vi "main-thermocouple-logger.vi"() -> ()   [LabVIEW 2024]
uses:
  controls/adam-5000-serial-settings.ctl
  controls/adam-5000-cmd-response.ctl
  controls/state-enum.ctl
  sub-vi/csv-file-logging/filepath-selection.ctl
  controls/adam-5000-all-chassis-data.ctl
  controls/adam-5000-all-module-datas.ctl
  controls/digital-output-cluster.ctl
  controls/digitial-input-cluster.ctl
  controls/analog-output-cluster.ctl
  controls/analog-input-cluster.ctl
  controls/thermocouple-input-cluster.ctl
  controls/adam-5000-chassis-cmd-ack.ctl
  controls/adam-5000-chassis-module-types.ctl
  controls/adam-5000-DO-user-input.ctl
  controls/adam-5000-status-indicator-references.ctl
panel:
  out "T12":dbl
  out "T11":dbl
  out "T6 (Airgap)":dbl
  out "T5 (Ambi)":dbl
  in  "TC5:8 Zero Point Offset":cluster{"T5":dbl, "T6":dbl, "T7":dbl, "T8":dbl}
  in  "TC1:4 Zero point offset":cluster{"T1":dbl, "T2":dbl, "T3":dbl, "T4":dbl}
  in  "Calibration":bool
  in  "clear-graphs":bool
  out "Thermocouples 5-8":T1(graph)
  out "Thermocouples 1-4":T1(graph)
  out "T10":dbl
  out "T9":dbl
  out "T8":dbl
  out "T7":dbl
  out "T4":dbl
  out "T3":dbl
  out "T2":dbl
  out "T1":dbl
  out "Hz":dbl format="%_3g"
  in  "Sample Rate (Hz)":dbl=1.0 min=0.0001 max=4.0 format="%#_4g"
  out "Logged Data String":string
  in  "CSV Data Headings":string="time (s),T1,T2,T3,T4,T5(Ambi),T6(Airgap),T7, T8, T9, T10, T11, T12"
  out "log-elapsed time":dbl format="%.2f"
  out "log start time":u32
  out "File Open":bool
  out "Log Filepath":path
  in  "Log Filepath Selection":T2={"Log Filepath Source"=enum."Application Relative (Auto)", "Log File Path (Manual)"=path "C:/Users/iwheard/Documents/0000-labview/adam5000-generic-controller/data", "Log File Folder Name"="data", "log file name"="log", "Include Date in Filename"=TRUE, "Include Time in Filename"=TRUE}
  out "Logging Active":bool
  out "Error Detected":bool
  in  "Reset":bool
  out "ADAM Connected":bool
  in  "Stop ADAM":bool
  in  "Start Logging":bool
  out "Program State":T3
  in  "Start ADAM":bool
  out "cmd-response":T5
  out "Status Indicators":T6
  in  "Debug Mode":bool
  in  "Chassis Settings":T7={"VISA resource name"="COM3", "baud rate (19200)"=19200, "Chassis ID"=1}
  out "Loop Time (mS)":u32
  out "Loop Counter":i32
  out "error":errorcluster
  in  "exit":bool
  # "ADAM 5000 Controller"
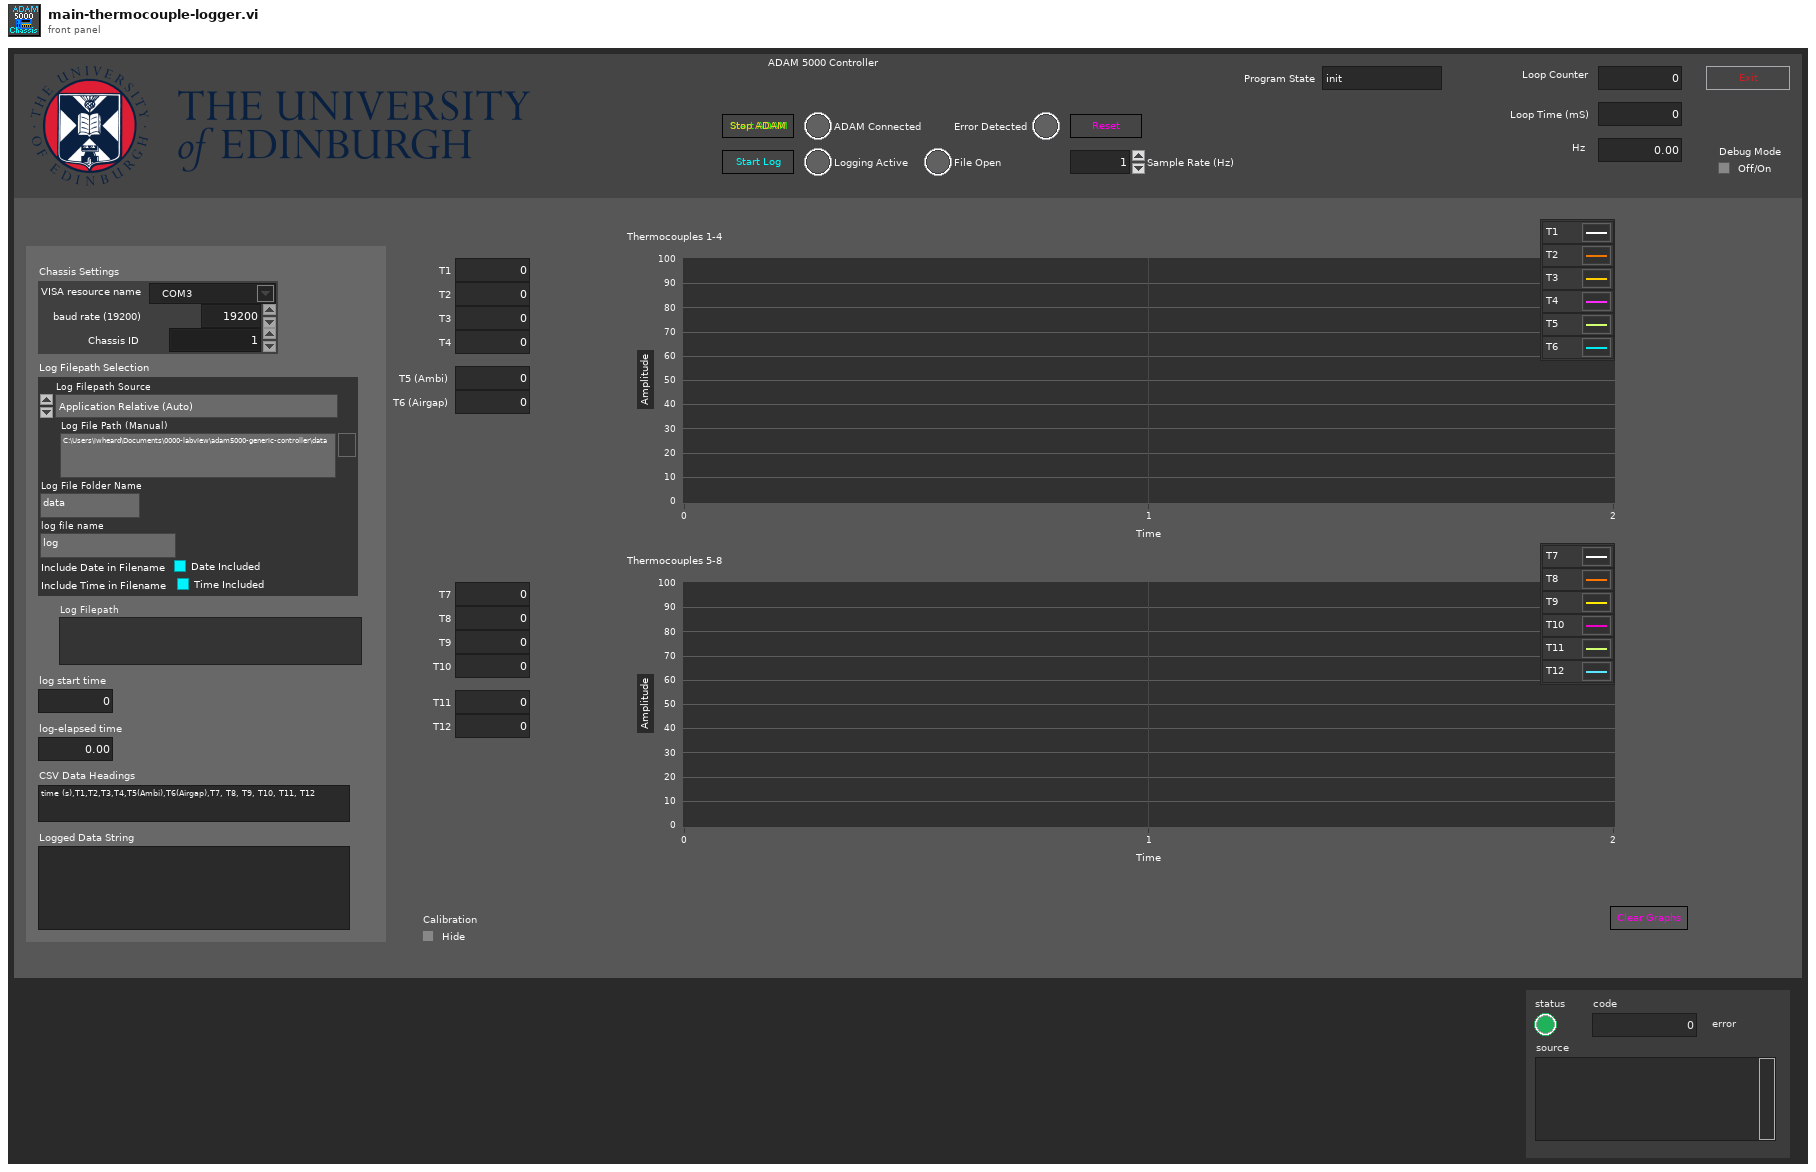
[diagram p1: front panel]
types:
  T1 = cluster{"TC0":dbl, "TC1":dbl, "TC2":dbl, "TC3":dbl, "TC4":dbl, "TC5":dbl, "TC6":dbl}
  T2 = typedef "filepath-selection.ctl" = cluster{"Log Filepath Source":enum16{"Application Relative (Auto)", "VI Relative (Auto)", "Complete Path (Manual)"}, "Log File Path (Manual)":path, "Log File Folder Name":string, "log file name":string, "Include Date in Filename":bool, "Include Time in Filename":bool}
  T3 = typedef "state-enum.ctl" = enum16{"init", "wait", "manual", "start", "run", "reset", "stop", "exit"}
  T4 = typedef "adam-5000-cmd-response.ctl" = cluster{"cmd string":string, "response":string}
  T5 = cluster{"cmd-response:0":T4, "cmd-response:1":T4, "cmd-response:2":T4, "cmd-response:3":T4, "cmd-response:4":T4, "cmd-response:5":T4, "cmd-response:6":T4, "cmd-response:7":T4}
  T6 = cluster{"status-indicator:0":cluster{"Sampling":bool, "Ack":bool}, "status-indicator:1":cluster{"Sampling":bool, "Ack":bool}, "status-indicator:2":cluster{"Sampling":bool, "Ack":bool}, "status-indicator:3":cluster{"Sampling":bool, "Ack":bool}, "status-indicator:4":cluster{"Sampling":bool, "Ack":bool}, "status-indicator:5":cluster{"Sampling":bool, "Ack":bool}, "status-indicator:6":cluster{"Sampling":bool, "Ack":bool}, "status-indicator:7":cluster{"Sampling":bool, "Ack":bool}}
  T7 = typedef "adam-5000-serial-settings.ctl" = cluster{"VISA resource name":refnum<visa-resource-name>, "baud rate (19200)":u32, "Chassis ID":u8}
  T8 = enum16{"Digital Output", "Digital Input", "Analog Output", "Analog Input", "Thermocouple", "Power Relay", "empty"}
  T9 = typedef "adam-5000-chassis-module-types.ctl" = cluster{"Slot 0: Module Type":enum16{"Digital Output", "Digital Input", "Analog Output", "Analog Input", "Thermocouple", "Power Relay", "empty"}, "Slot 1: Module Type":enum16{"Digital Output", "Digital Input", "Analog Output", "Analog Input", "Thermocouple", "Power Relay", "empty"}, "Slot 2: Module Type":enum16{"Digital Output", "Digital Input", "Analog Output", "Analog Input", "Thermocouple", "Power Relay", "empty"}, "Slot 3: Module Type":enum16{"Digital Output", "Digital Input", "Analog Output", "Analog Input", "Thermocouple", "Power Relay", "empty"}, "Slot 4: Module Type":enum16{"Digital Output", "Digital Input", "Analog Output", "Analog Input", "Thermocouple", "Power Relay", "empty"}, "Slot 5: Module Type":enum16{"Digital Output", "Digital Input", "Analog Output", "Analog Input", "Thermocouple", "Power Relay", "empty"}, "Slot 6: Module Type":enum16{"Digital Output", "Digital Input", "Analog Output", "Analog Input", "Thermocouple", "Power Relay", "empty"}, "Slot 7: Module Type":enum16{"Digital Output", "Digital Input", "Analog Output", "Analog Input", "Thermocouple", "Power Relay", "empty"}}
  T10 = typedef "adam-5000-chassis-cmd-ack.ctl" = cluster{"cmd-response:0":T4, "cmd-response:1":T4, "cmd-response:2":T4, "cmd-response:3":T4, "cmd-response:4":T4, "cmd-response:5":T4, "cmd-response:6":T4, "cmd-response:7":T4}
  T11 = typedef "adam-5000-all-chassis-data.ctl" = cluster{"slot:0":T12, "slot:1":T12, "slot:2":T12, "slot:3":T12, "slot:4":T12, "slot:5":T12, "slot:6":T12, "slot:7":T12}
  T12 = typedef "adam-5000-all-module-datas.ctl" = cluster{"Digital Outputs":T13, "Digital Inputs":T14, "Analog Outputs":T15, "Analog Inputs":T16, "Thermocouple Inputs (degC)":T17}
  T13 = typedef "digital-output-cluster.ctl" = cluster{"DO0":bool, "DO1":bool, "DO2":bool, "DO3":bool, "DO4":bool, "DO5":bool, "DO6":bool, "DO7":bool}
  T14 = typedef "digitial-input-cluster.ctl" = cluster{"DI0":bool, "DI1":bool, "DI2":bool, "DI3":bool, "DI4":bool, "DI5":bool, "DI6":bool, "DI7":bool}
  T15 = typedef "analog-output-cluster.ctl" = cluster{"AO0":dbl, "AO1":dbl, "AO2":dbl, "AO3":dbl}
  T16 = typedef "analog-input-cluster.ctl" = cluster{"AI0":dbl, "AI1":dbl, "AI2":dbl, "AI3":dbl, "AI4":dbl, "AI5":dbl, "AI6":dbl, "AI7":dbl}
  T17 = typedef "thermocouple-input-cluster.ctl" = cluster{"TC0":dbl, "TC1":dbl, "TC2":dbl, "TC3":dbl, "TC4":dbl, "TC5":dbl, "TC6":dbl}
  T18 = enum8{"Enabled", "Disabled", "Disabled and Grayed Out"}
  T19 = typedef "adam-5000-status-indicator-references.ctl" = cluster{"status-indicator:0":refnum<vi>, "status-indicator:1":refnum<vi>, "status-indicator:2":refnum<vi>, "status-indicator:3":refnum<vi>, "status-indicator:4":refnum<vi>, "status-indicator:5":refnum<vi>, "status-indicator:6":refnum<vi>, "status-indicator:7":refnum<vi>}
  T20 = typedef "adam-5000-DO-user-input.ctl" = cluster{"0:Digital Outputs":T13, "1:Digital Outputs":T13, "2:Digital Outputs":T13, "3:Digital Outputs":T13, "4:Digital Outputs":T13, "5:Digital Outputs":T13, "6:Digital Outputs":T13, "7:Digital Outputs":T13}
  T21 = cluster{"TC0":dbl, "TC1":dbl, "TC2":dbl, "TC3":dbl, "TC4":dbl, "TC5":dbl, "TC6":dbl}[]
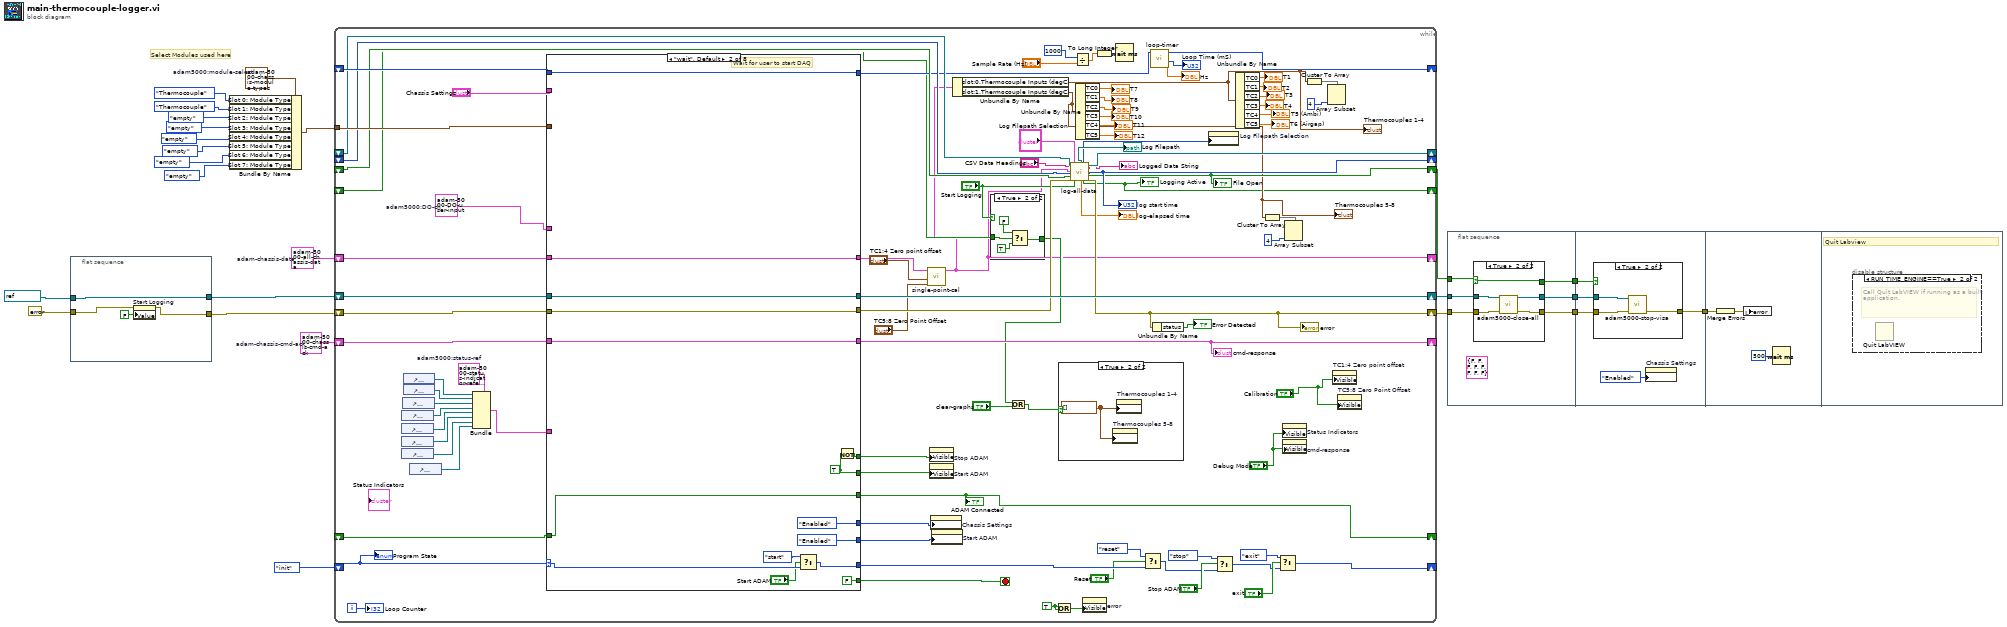
[diagram p0: block diagram]
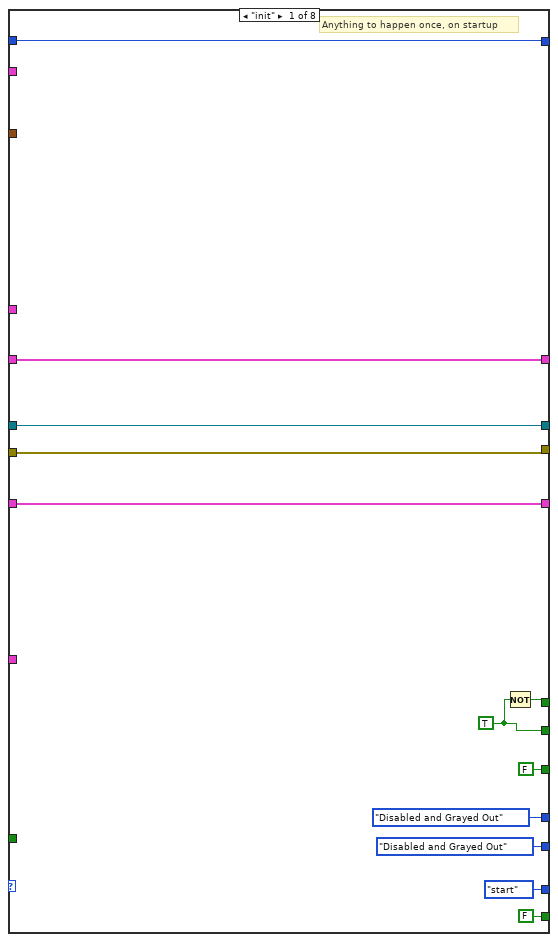
[diagram p7: hidden frame]
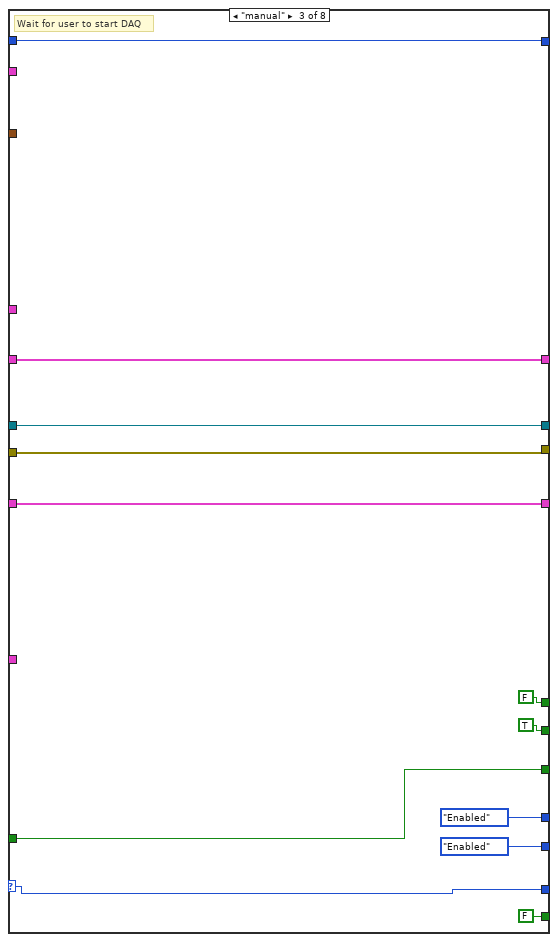
[diagram p8: hidden frame]
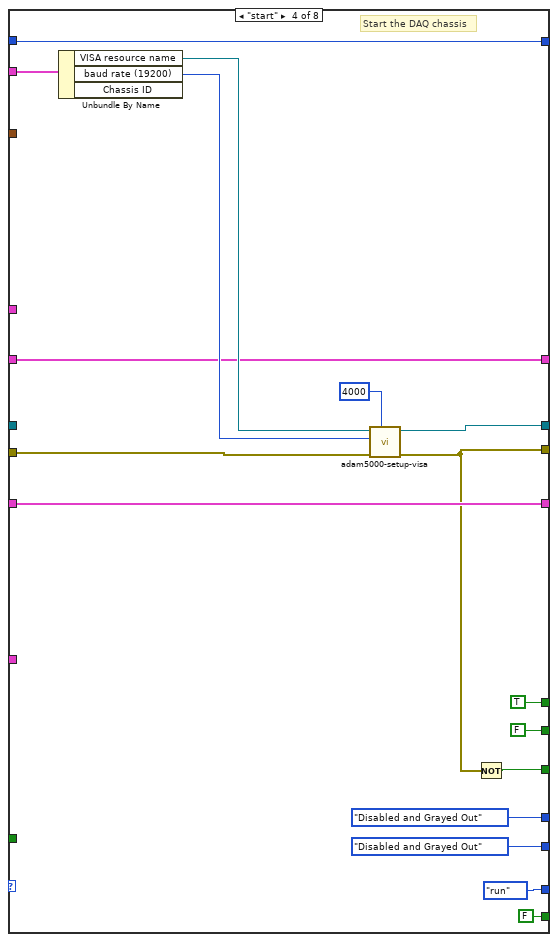
[diagram p9: hidden frame]
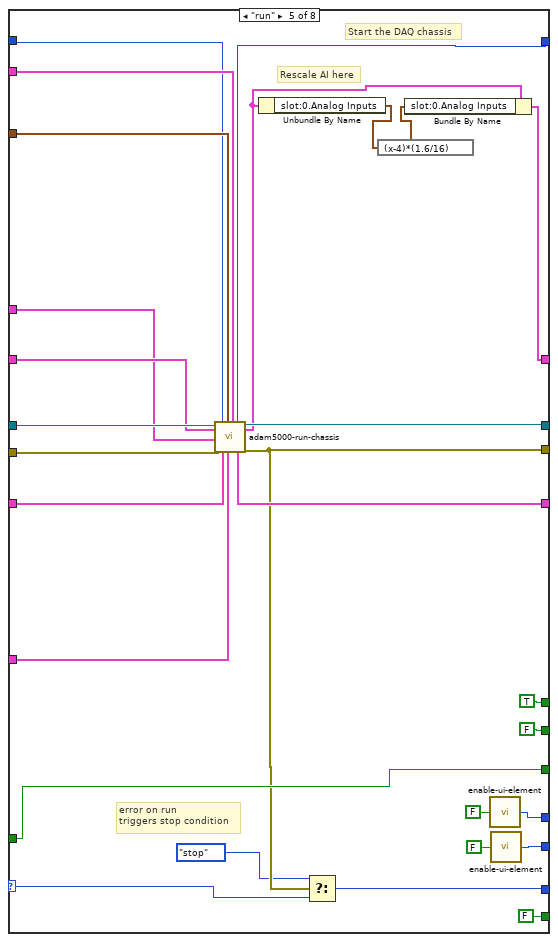
[diagram p10: hidden frame]
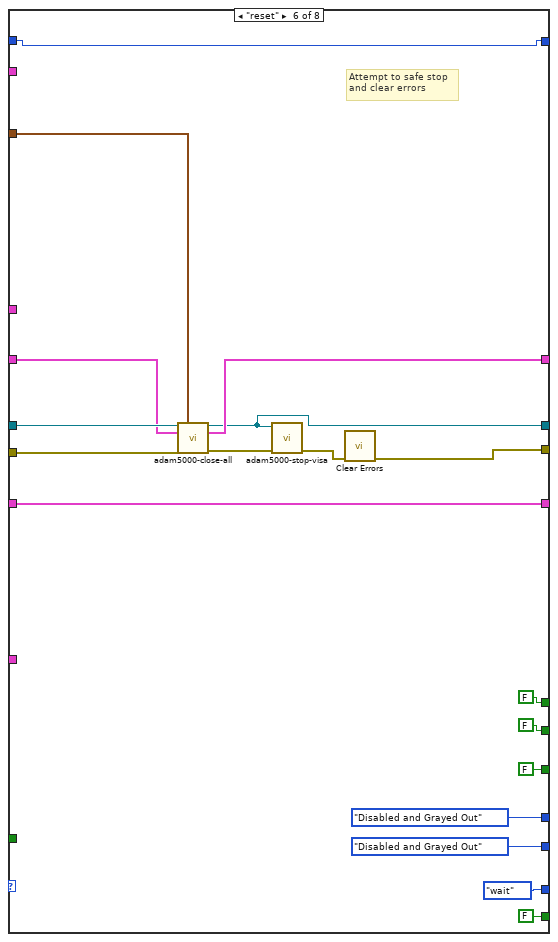
[diagram p11: hidden frame]
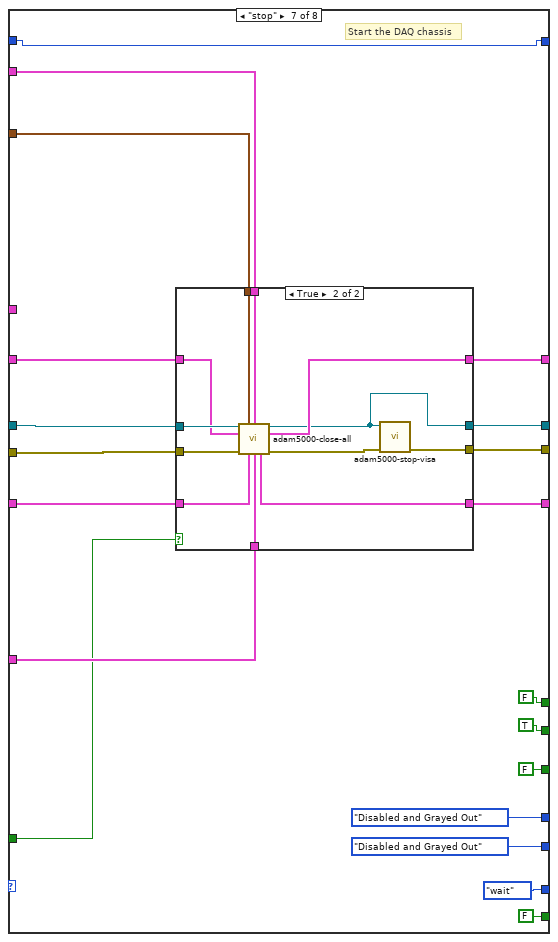
[diagram p12: hidden frame]
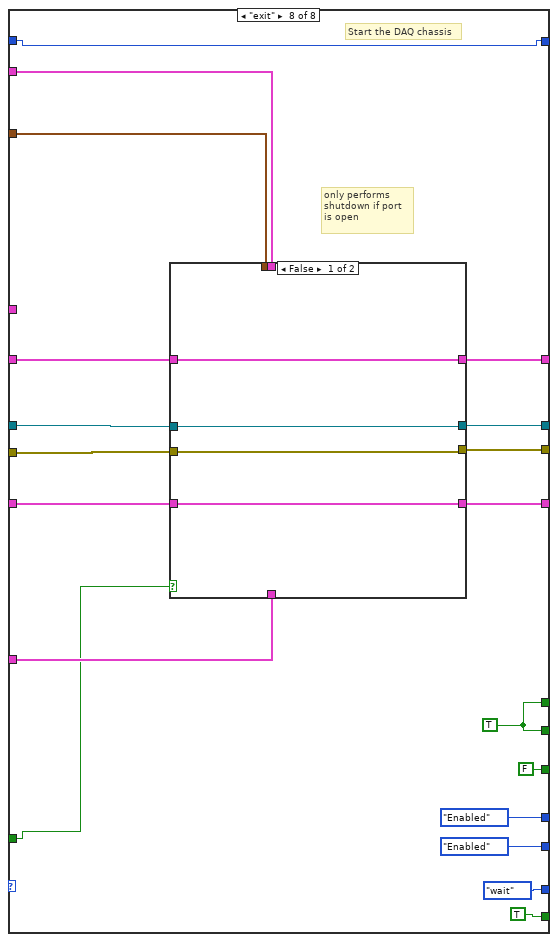
[diagram p14: hidden frame]
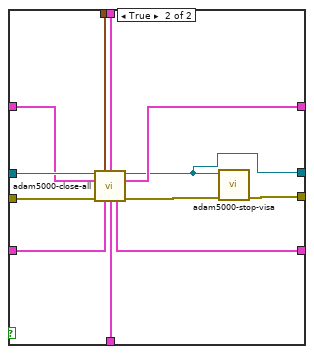
[diagram p15: hidden frame]
diagram:
  w16 = T9 {"Slot 0: Module Type"=enum."Digital Output", "Slot 1: Module Type"=enum."Digital Output", "Slot 2: Module Type"=enum."Digital Output", "Slot 3: Module Type"=enum."Digital Output", "Slot 4: Module Type"=enum."Digital Output", "Slot 5: Module Type"=enum."Digital Output", "Slot 6: Module Type"=enum."Digital Output", "Slot 7: Module Type"=enum."Digital Output"}  # adam5000:module-select
  w21 = T10 {"cmd-response:0"={"cmd string"="", "response"=""}, "cmd-response:1"={"cmd string"="", "response"=""}, "cmd-response:2"={"cmd string"="", "response"=""}, "cmd-response:3"={"cmd string"="", "response"=""}, "cmd-response:4"={"cmd string"="", "response"=""}, "cmd-response:5"={"cmd string"="", "response"=""}, "cmd-response:6"={"cmd string"="", "response"=""}, "cmd-response:7"={"cmd string"="", "response"=""}}  # adam-chassis-cmd-ack
  w22 = T11 {"slot:0"={"Digital Outputs"={"DO0"=FALSE, "DO1"=FALSE, "DO2"=FALSE, "DO3"=FALSE, "DO4"=FALSE, "DO5"=FALSE, "DO6"=FALSE, "DO7"=FALSE}, "Digital Inputs"={"DI0"=FALSE, "DI1"=FALSE, "DI2"=FALSE, "DI3"=FALSE, "DI4"=FALSE, "DI5"=FALSE, "DI6"=FALSE, "DI7"=FALSE}, "Analog Outputs"={"AO0"=0.0, "AO1"=0.0, "AO2"=0.0, "AO3"=0.0}, "Analog Inputs"={"AI0"=0.0, "AI1"=0.0, "AI2"=0.0, "AI3"=0.0, "AI4"=0.0, "AI5"=0.0, "AI6"=0.0, "AI7"=0.0}, "Thermocouple Inputs (degC)"={"TC0"=0.0, "TC1"=0.0, "TC2"=0.0, "TC3"=0.0, "TC4"=0.0, "TC5"=0.0, "TC6"=0.0}}, "slot:1"={"Digital Outputs"={"DO0"=FALSE, "DO1"=FALSE, "DO2"=FALSE, "DO3"=FALSE, "DO4"=FALSE, "DO5"=FALSE, "DO6"=FALSE, "DO7"=FALSE}, "Digital Inputs"={"DI0"=FALSE, "DI1"=FALSE, "DI2"=FALSE, "DI3"=FALSE, "DI4"=FALSE, "DI5"=FALSE, "DI6"=FALSE, "DI7"=FALSE}, "Analog Outputs"={"AO0"=0.0, "AO1"=0.0, "AO2"=0.0, "AO3"=0.0}, "Analog Inputs"={"AI0"=0.0, "AI1"=0.0, "AI2"=0.0, "AI3"=0.0, "AI4"=0.0, "AI5"=0.0, "AI6"=0.0, "AI7"=0.0}, "Thermocouple Inputs (degC)"={"TC0"=0.0, "TC1"=0.0, "TC2"=0.0, "TC3"=0.0, "TC4"=0.0, "TC5"=0.0, "TC6"=0.0}}, "slot:2"={"Digital Outputs"={"DO0"=FALSE, "DO1"=FALSE, "DO2"=FALSE, "DO3"=FALSE, "DO4"=FALSE, "DO5"=FALSE, "DO6"=FALSE, "DO7"=FALSE}, "Digital Inputs"={"DI0"=FALSE, "DI1"=FALSE, "DI2"=FALSE, "DI3"=FALSE, "DI4"=FALSE, "DI5"=FALSE, "DI6"=FALSE, "DI7"=FALSE}, "Analog Outputs"={"AO0"=0.0, "AO1"=0.0, "AO2"=0.0, "AO3"=0.0}, "Analog Inputs"={"AI0"=0.0, "AI1"=0.0, "AI2"=0.0, "AI3"=0.0, "AI4"=0.0, "AI5"=0.0, "AI6"=0.0, "AI7"=0.0}, "Thermocouple Inputs (degC)"={"TC0"=0.0, "TC1"=0.0, "TC2"=0.0, "TC3"=0.0, "TC4"=0.0, "TC5"=0.0, "TC6"=0.0}}, "slot:3"={"Digital Outputs"={"DO0"=FALSE, "DO1"=FALSE, "DO2"=FALSE, "DO3"=FALSE, "DO4"=FALSE, "DO5"=FALSE, "DO6"=FALSE, "DO7"=FALSE}, "Digital Inputs"={"DI0"=FALSE, "DI1"=FALSE, "DI2"=FALSE, "DI3"=FALSE, "DI4"=FALSE, "DI5"=FALSE, "DI6"=FALSE, "DI7"=FALSE}, "Analog Outputs"={"AO0"=0.0, "AO1"=0.0, "AO2"=0.0, "AO3"=0.0}, "Analog Inputs"={"AI0"=0.0, "AI1"=0.0, "AI2"=0.0, "AI3"=0.0, "AI4"=0.0, "AI5"=0.0, "AI6"=0.0, "AI7"=0.0}, "Thermocouple Inputs (degC)"={"TC0"=0.0, "TC1"=0.0, "TC2"=0.0, "TC3"=0.0, "TC4"=0.0, "TC5"=0.0, "TC6"=0.0}}, "slot:4"={"Digital Outputs"={"DO0"=FALSE, "DO1"=FALSE, "DO2"=FALSE, "DO3"=FALSE, "DO4"=FALSE, "DO5"=FALSE, "DO6"=FALSE, "DO7"=FALSE}, "Digital Inputs"={"DI0"=FALSE, "DI1"=FALSE, "DI2"=FALSE, "DI3"=FALSE, "DI4"=FALSE, "DI5"=FALSE, "DI6"=FALSE, "DI7"=FALSE}, "Analog Outputs"={"AO0"=0.0, "AO1"=0.0, "AO2"=0.0, "AO3"=0.0}, "Analog Inputs"={"AI0"=0.0, "AI1"=0.0, "AI2"=0.0, "AI3"=0.0, "AI4"=0.0, "AI5"=0.0, "AI6"=0.0, "AI7"=0.0}, "Thermocouple Inputs (degC)"={"TC0"=0.0, "TC1"=0.0, "TC2"=0.0, "TC3"=0.0, "TC4"=0.0, "TC5"=0.0, "TC6"=0.0}}, "slot:5"={"Digital Outputs"={"DO0"=FALSE, "DO1"=FALSE, "DO2"=FALSE, "DO3"=FALSE, "DO4"=FALSE, "DO5"=FALSE, "DO6"=FALSE, "DO7"=FALSE}, "Digital Inputs"={"DI0"=FALSE, "DI1"=FALSE, "DI2"=FALSE, "DI3"=FALSE, "DI4"=FALSE, "DI5"=FALSE, "DI6"=FALSE, "DI7"=FALSE}, "Analog Outputs"={"AO0"=0.0, "AO1"=0.0, "AO2"=0.0, "AO3"=0.0}, "Analog Inputs"={"AI0"=0.0, "AI1"=0.0, "AI2"=0.0, "AI3"=0.0, "AI4"=0.0, "AI5"=0.0, "AI6"=0.0, "AI7"=0.0}, "Thermocouple Inputs (degC)"={"TC0"=0.0, "TC1"=0.0, "TC2"=0.0, "TC3"=0.0, "TC4"=0.0, "TC5"=0.0, "TC6"=0.0}}, "slot:6"={"Digital Outputs"={"DO0"=FALSE, "DO1"=FALSE, "DO2"=FALSE, "DO3"=FALSE, "DO4"=FALSE, "DO5"=FALSE, "DO6"=FALSE, "DO7"=FALSE}, "Digital Inputs"={"DI0"=FALSE, "DI1"=FALSE, "DI2"=FALSE, "DI3"=FALSE, "DI4"=FALSE, "DI5"=FALSE, "DI6"=FALSE, "DI7"=FALSE}, "Analog Outputs"={"AO0"=0.0, "AO1"=0.0, "AO2"=0.0, "AO3"=0.0}, "Analog Inputs"={"AI0"=0.0, "AI1"=0.0, "AI2"=0.0, "AI3"=0.0, "AI4"=0.0, "AI5"=0.0, "AI6"=0.0, "AI7"=0.0}, "Thermocouple Inputs (degC)"={"TC0"=0.0, "TC1"=0.0, "TC2"=0.0, "TC3"=0.0, "TC4"=0.0, "TC5"=0.0, "TC6"=0.0}}, "slot:7"={"Digital Outputs"={"DO0"=FALSE, "DO1"=FALSE, "DO2"=FALSE, "DO3"=FALSE, "DO4"=FALSE, "DO5"=FALSE, "DO6"=FALSE, "DO7"=FALSE}, "Digital Inputs"={"DI0"=FALSE, "DI1"=FALSE, "DI2"=FALSE, "DI3"=FALSE, "DI4"=FALSE, "DI5"=FALSE, "DI6"=FALSE, "DI7"=FALSE}, "Analog Outputs"={"AO0"=0.0, "AO1"=0.0, "AO2"=0.0, "AO3"=0.0}, "Analog Inputs"={"AI0"=0.0, "AI1"=0.0, "AI2"=0.0, "AI3"=0.0, "AI4"=0.0, "AI5"=0.0, "AI6"=0.0, "AI7"=0.0}, "Thermocouple Inputs (degC)"={"TC0"=0.0, "TC1"=0.0, "TC2"=0.0, "TC3"=0.0, "TC4"=0.0, "TC5"=0.0, "TC6"=0.0}}}  # adam-chassis-data
  # "Select Modules used here"
  n1 = flat-sequence {
    tunnel: [w27] -> w5
    tunnel: refnum<visa-resource-name> "COM8" ("VISA Refnum out") -> [w27]
    tunnel: errorcluster {"status"=FALSE, "code"=0, "source"=""} ("error in") -> [w26]
    tunnel: [w25] -> w3
    frame #0 {
      n2 = property on="Start Logging" class="Bool (strict)"(error in=w26, "Value"=FALSE ("Start Logging")) -> (error out=w25:errorcluster)  [unwired: 1 in, 1 out]
    }
  }
  n3 = Bundle By Name(cluster=w16, "Slot 0: Module Type"=T8."Thermocouple", "Slot 1: Module Type"=T8."Thermocouple", "Slot 2: Module Type"=T8."empty" ("Slot 1: Module Type"), "Slot 3: Module Type"=T8."empty" ("Slot 1: Module Type"), "Slot 4: Module Type"=T8."empty" ("Slot 1: Module Type"), "Slot 5: Module Type"=T8."empty" ("Slot 1: Module Type"), "Slot 6: Module Type"=T8."empty" ("Slot 1: Module Type"), "Slot 7: Module Type"=T8."empty" ("Slot 1: Module Type")) -> (w7:T9)
  n4 = while {
    shift-right: [w101] -> _
    shift-left: state-enum."init" ("state-enum") -> [w84]
    shift-right: [w67] -> _
    shift-left: _ -> [w105]
    shift-right: [w93] -> w20
    shift-left: w5 -> [w108]
    shift-right: [w71] -> w19
    shift-left: w3 -> [w107]
    shift-right: [w35] -> _
    shift-left: w22 -> [w104]
    shift-right: [w86] -> _
    shift-left: w21 -> [w103]
    shift-right: [w91] -> _
    shift-left: _ -> [w92]
    tunnel: w7 -> [w85]
    shift-right: [w59] -> w2
    shift-left: _ -> [w72]
    shift-right: [w60] -> _
    shift-left: _ -> [w73]
    shift-right: [w77] -> _
    shift-left: _ -> [w80]
    shift-right: [w43] -> _
    shift-left: _ -> [w39]
    i -> [w122]
    stop <- w94 stop-if-true
    w112 = T19 {"status-indicator:0"=refnum, "status-indicator:1"=refnum, "status-indicator:2"=refnum, "status-indicator:3"=refnum, "status-indicator:4"=refnum, "status-indicator:5"=refnum, "status-indicator:6"=refnum, "status-indicator:7"=refnum}  # adam5000:status-ref
    w58 = T20 {"0:Digital Outputs"={"DO0"=FALSE, "DO1"=FALSE, "DO2"=FALSE, "DO3"=FALSE, "DO4"=FALSE, "DO5"=FALSE, "DO6"=FALSE, "DO7"=FALSE}, "1:Digital Outputs"={"DO0"=FALSE, "DO1"=FALSE, "DO2"=FALSE, "DO3"=FALSE, "DO4"=FALSE, "DO5"=FALSE, "DO6"=FALSE, "DO7"=FALSE}, "2:Digital Outputs"={"DO0"=FALSE, "DO1"=FALSE, "DO2"=FALSE, "DO3"=FALSE, "DO4"=FALSE, "DO5"=FALSE, "DO6"=FALSE, "DO7"=FALSE}, "3:Digital Outputs"={"DO0"=FALSE, "DO1"=FALSE, "DO2"=FALSE, "DO3"=FALSE, "DO4"=FALSE, "DO5"=FALSE, "DO6"=FALSE, "DO7"=FALSE}, "4:Digital Outputs"={"DO0"=FALSE, "DO1"=FALSE, "DO2"=FALSE, "DO3"=FALSE, "DO4"=FALSE, "DO5"=FALSE, "DO6"=FALSE, "DO7"=FALSE}, "5:Digital Outputs"={"DO0"=FALSE, "DO1"=FALSE, "DO2"=FALSE, "DO3"=FALSE, "DO4"=FALSE, "DO5"=FALSE, "DO6"=FALSE, "DO7"=FALSE}, "6:Digital Outputs"={"DO0"=FALSE, "DO1"=FALSE, "DO2"=FALSE, "DO3"=FALSE, "DO4"=FALSE, "DO5"=FALSE, "DO6"=FALSE, "DO7"=FALSE}, "7:Digital Outputs"={"DO0"=FALSE, "DO1"=FALSE, "DO2"=FALSE, "DO3"=FALSE, "DO4"=FALSE, "DO5"=FALSE, "DO6"=FALSE, "DO7"=FALSE}}  # adam5000:DO-ch
    w95 = TRUE ("Debug Mode")
    n5 = control-ref of="status-indicator:4"() -> (w116:refnum<vi>)
    n6 = control-ref of="status-indicator:5"() -> (w115:refnum<vi>)
    n7 = control-ref of="status-indicator:3"() -> (w117:refnum<vi>)
    n8 = control-ref of="status-indicator:6"() -> (w114:refnum<vi>)
    n9 = control-ref of="status-indicator:2"() -> (w118:refnum<vi>)
    n10 = control-ref of="status-indicator:0"() -> (w120:refnum<vi>)
    n11 = control-ref of="status-indicator:1"() -> (w119:refnum<vi>)
    n12 = control-ref of="status-indicator:7"() -> (w113:refnum<vi>)
    n13 = Bundle(cluster=w112, "status-indicator:0"=w120, "status-indicator:1"=w119, "status-indicator:2"=w118, "status-indicator:3"=w117, "status-indicator:4"=w116, "status-indicator:5"=w115, "status-indicator:6"=w114, "status-indicator:7"=w113) -> (w102:T19)
    n14 = case shown="\"wait\", Default" w84 {
      selector: w84 -> [_ w153 w163 _ w197 _ _ _]
      tunnel: [state-enum."start" ("state-enum") w154 w163 state-enum."run" ("state-enum") w198 state-enum."wait" ("state-enum") state-enum."wait" ("state-enum") state-enum."wait" ("state-enum")] -> w89
      tunnel: [T18."Disabled and Grayed Out" ("Disabled") T18."Enabled" ("Disabled") T18."Enabled" ("Disabled") T18."Disabled and Grayed Out" ("Disabled") w187 T18."Disabled and Grayed Out" ("Disabled") T18."Disabled and Grayed Out" ("Disabled") T18."Enabled" ("Disabled")] -> w110
      tunnel: [T18."Disabled and Grayed Out" ("Disabled") T18."Enabled" ("Disabled") T18."Enabled" ("Disabled") T18."Disabled and Grayed Out" ("Disabled") w185 T18."Disabled and Grayed Out" ("Disabled") T18."Disabled and Grayed Out" ("Disabled") T18."Enabled" ("Disabled")] -> w109
      tunnel: w108 -> [w137 w150 w165 _ w212 w221 w247 w282]
      tunnel: [w137 w150 w165 w182 w210 w215 w237 w270] -> w93
      tunnel: w107 -> [w136 w149 w164 w181 w211 w220 w246 w281]
      tunnel: [w136 w149 w164 w171 w196 w224 w236 w271] -> w70
      tunnel: "Chassis Settings" -> [_ _ _ w180 w209 _ w244 w279]
      tunnel: w85 -> [_ _ _ _ w208 w217 w245 w280]
      tunnel: w105 -> [w135 w147 w162 w175 w207 w226 w238 w273]
      tunnel: [w135 w147 w162 w175 w206 w226 w238 w273] -> w68
      tunnel: w104 -> [w134 w146 w161 w174 w205 w219 w243 w278]
      tunnel: w58 -> [_ _ _ _ w204 _ _ _]
      tunnel: w103 -> [w133 w145 w160 w173 w203 w225 w241 w276]
      tunnel: w102 -> [_ _ _ _ w202 _ w240 w275]
      tunnel: [w133 w145 w160 w173 w201 w225 w239 w274] -> w86
      tunnel: [w134 w146 w161 w174 w191 w218 w242 w277] -> w37
      tunnel: [FALSE FALSE FALSE FALSE FALSE FALSE FALSE TRUE] -> w94
      tunnel: [FALSE w143 w158 w170 w199 FALSE FALSE FALSE] -> w91
      tunnel: w92 -> [_ w143 w158 _ w199 _ w233 w268]
      tunnel: [w130 w141 TRUE ("Visible") FALSE ("Visible") FALSE ("Visible") FALSE ("Visible") TRUE ("Visible") w267] -> w83
      tunnel: [w129 w142 FALSE ("Visible") TRUE ("Visible") TRUE ("Visible") FALSE ("Visible") FALSE ("Visible") w267] -> w82
      frame "init" {
        w130 = TRUE ("Visible")
        # "Anything to happen once, on startup"
        n15 = Not(x=w130) -> (.not. x?=w129:bool)
      }
      frame "wait", Default {
        w141 = TRUE ("Visible")
        # "Wait for user to start DAQ"
        n16 = Select(t=state-enum."start" ("state-enum"), s="Start ADAM", f=w153) -> (s? t:f=w154:T3)
        n17 = Not(x=w141) -> (.not. x?=w142:bool)
      }
      frame "manual" {
        # "Wait for user to start DAQ"
      }
      frame "start" {
        # "Start the DAQ chassis"
        n18 = Unbundle By Name(w180) -> ("VISA resource name"=w179:refnum<visa-resource-name>, "baud rate (19200)"=w178:u32)  [unwired: 1 out]
        n19 = call "adam5000-setup-visa.vi"("timeout (10sec)"=u32 4000, "error in"=w181, "baud rate (19200)"=w178, "VISA Refnum in"=w179) -> ("error out"=w171:errorcluster, "VISA Refnum out"=w182:refnum<visa-resource-name>)  [unwired: 6 in]
        n20 = Not(x=w171) -> (.not. x?=w170:bool)
      }
      frame "run" {
        # "Rescale AI here"
        # "error on run\ntriggers stop condition"
        # "Start the DAQ chassis"
        n21 = call "adam5000-run-chassis.vi"("VISA Refnum In"=w212, "adam-chassis-all-data-in"=w205, "adam-chassis-all-DO-in"=w204, "error in"=w211, "loop-time-in"=w207, "adam-chassis-cmd-response-in"=w203, "adam-chassis-module-select-in"=w208, "adam5000:status-ref-in"=w202, "Chassis Settings"=w209) -> ("loop-time-out"=w206:u32, "adam-chassis-cmd-response-out"=w201:T10, "VISA Refnum Out"=w210:refnum<visa-resource-name>, "adam-chassis-all-data-out"=w192:T11, "error out"=w196:errorcluster)  [unwired: 5 in, 1 out]
        n22 = Unbundle By Name(w192) -> ("slot:0.Analog Inputs"=w190:T16)
        n23 = Select(t=state-enum."stop", s=w196, f=w197) -> (s? t:f=w198:T3)
        n24 = expression code="(x-4)*(1.6/16)"(w190) -> (w189:T16)
        n25 = Bundle By Name(cluster=w192, "slot:0.Analog Inputs"=w189) -> (w191:T11)
        n26 = call "enable-ui-element.vi"("Enable UI Element"=FALSE) -> ("UI Element State"=w187:T18)  [unwired: 8 in]
        n27 = call "enable-ui-element.vi"("Enable UI Element"=FALSE) -> ("UI Element State"=w185:T18)  [unwired: 8 in]
      }
      frame "reset" {
        # "Attempt to safe stop\nand clear errors"
        n28 = call "adam5000-close-all.vi"("VISA Refnum in"=w221, "adam5000:module-type-select"=w217, "adam5000:all-data-in"=w219, "error in (no error)"=w220) -> ("VISA Refnum out"=w215:refnum<visa-resource-name>, "adam5000:all-data-out"=w218:T11, "error out"=w222:errorcluster)  [unwired: 8 in, 1 out]
        n29 = call "adam5000-stop-visa.vi"("error in (no error)"=w222, "VISA resource in"=w215) -> ("error out"=w216:errorcluster)  [unwired: 9 in]
        n30 = call <vilib>:"Clear Errors.vi"("error in (no error)"=w216) -> ("error out"=w224:errorcluster)  [unwired: 5 in, 1 out]
      }
      frame "stop" {
        # "Start the DAQ chassis"
        n31 = case shown="True" w233 {
          tunnel: w247 -> [w252 w266]
          tunnel: w246 -> [w251 w265]
          tunnel: w245 -> [_ w264]
          tunnel: w244 -> [_ w263]
          tunnel: w243 -> [w254 w262]
          tunnel: [w254 w261] -> w242
          tunnel: w241 -> [w253 w260]
          tunnel: w240 -> [_ w259]
          tunnel: [w253 w258] -> w239
          tunnel: [w252 w257] -> w237
          tunnel: [w251 w255] -> w236
          frame False {
          }
          frame True {
            n32 = call "adam5000-close-all.vi"("VISA Refnum in"=w266, "adam5000:module-type-select"=w264, "Chassis Settings in"=w263, "adam5000:all-data-in"=w262, "error in (no error)"=w265, "adam-chassis-cmd-ack"=w260, "adam5000:status-ref"=w259) -> ("VISA Refnum out"=w257:refnum<visa-resource-name>, "adam5000:all-data-out"=w261:T11, "adam-chassis-cmd-response-out"=w258:T10, "error out"=w256:errorcluster)  [unwired: 5 in]
            n33 = call "adam5000-stop-visa.vi"("error in (no error)"=w256, "VISA resource in"=w257) -> ("error out"=w255:errorcluster)  [unwired: 9 in]
          }
        }
      }
      frame "exit" {
        w267 = TRUE ("Visible")
        # "only performs\nshutdown if port\nis open"
        # "Start the DAQ chassis"
        n34 = case shown="False" w268 {
          tunnel: w282 -> [w288 w301]
          tunnel: w281 -> [w287 w300]
          tunnel: w280 -> [_ w299]
          tunnel: w279 -> [_ w298]
          tunnel: w278 -> [w289 w297]
          tunnel: [w289 w296] -> w277
          tunnel: w276 -> [w286 w295]
          tunnel: w275 -> [_ w294]
          tunnel: [w286 w293] -> w274
          tunnel: [w287 w291] -> w271
          tunnel: [w288 w290] -> w270
          frame False {
          }
          frame True {
            n35 = call "adam5000-close-all.vi"("VISA Refnum in"=w301, "adam5000:module-type-select"=w299, "Chassis Settings in"=w298, "adam5000:all-data-in"=w297, "error in (no error)"=w300, "adam-chassis-cmd-ack"=w295, "adam5000:status-ref"=w294) -> ("VISA Refnum out"=w290:refnum<visa-resource-name>, "adam5000:all-data-out"=w296:T11, "adam-chassis-cmd-response-out"=w293:T10, "error out"=w292:errorcluster)  [unwired: 5 in]
            n36 = call "adam5000-stop-visa.vi"("error in (no error)"=w292, "VISA resource in"=w290) -> ("error out"=w291:errorcluster)  [unwired: 9 in]
          }
        }
      }
    }
    "cmd-response" <- w86
    "ADAM Connected" <- w91
    n37 = call "single-point-cal.vi"("TC5:8 Zero Point Offset"="TC5:8 Zero Point Offset", "TC1:4 Zero point offset"="TC1:4 Zero point offset", "adam5000:all-data-in"=w37) -> ("adam5000:all-data-out"=w35:T11)  [unwired: 8 in]
    n38 = property on="Stop ADAM" class="Bool"("Visible"=w82) -> ()  [unwired: 2 in, 2 out]
    n39 = property on="Start ADAM" class="Bool"("Visible"=w83) -> ()  [unwired: 2 in, 2 out]
    n40 = property on="Chassis Settings" class="Clust (strict)"("DisabledEnum"=w110) -> ()  [unwired: 2 in, 2 out]
    n41 = property on="Start ADAM" class="Bool"("DisabledEnum"=w109) -> ()  [unwired: 2 in, 2 out]
    n42 = Unbundle By Name(w35) -> ("slot:0.Thermocouple Inputs (degC)"=w45:T17, "slot:1.Thermocouple Inputs (degC)"=w44:T17)
    "Thermocouples 1-4" <- w45
    "Thermocouples 5-8" <- w44
    n43 = case shown="True" "Start Logging" {
      selector: "Start Logging" -> [w123 _]
      tunnel: w39 -> [_ w127]
      tunnel: [w123 w125] -> w38
      frame False {
      }
      frame True {
        n44 = Select(t=FALSE ("Visible"), s=w127, f=TRUE ("Visible")) -> (s? t:f=w125:bool)
      }
    }
    n45 = Or(x=w38, y="clear-graphs") -> (x .or. y?=w42:bool)
    n46 = Or(x=w95, y=w95) -> (x .or. y?=w121:bool)
    n47 = case shown="True" w42 {
      frame False {
      }
      frame True {
        w128 = T21 [] ("History Data")
        n48 = property on="Thermocouples 5-8" class="WFChart (strict)"("History Data"=w128) -> ()  [unwired: 2 in, 2 out]
        n49 = property on="Thermocouples 1-4" class="WFChart (strict)"("History Data"=w128) -> ()  [unwired: 2 in, 2 out]
      }
    }
    n50 = call "log-all-data.vi"("log-file-byte-stream"=w80, "CSV Data Headings"="CSV Data Headings", "adam5000:all-data-in"=w35, "log-start-time(mS)"=w73, "file open?"=w72, "error in (no error)"=w70, "Log Filepath Selection"="Log Filepath Selection", "Start Logging"="Start Logging") -> ("appended path for log file"=→"Log Filepath":path, "log-elapsed time"=→"log-elapsed time":dbl, "log-filepath-enable-state"=w76:T18, "Start Logging"=w43:bool, "log-file-bytestream"=w77:refnum<file>, "Logged Data String"=→"Logged Data String":string, "log-start-time(mS)"=w60:u32, "file open?"=w59:bool, "error out"=w71:errorcluster)  [unwired: 3 in]
    "error" <- w71
    "Logging Active" <- w43
    "File Open" <- w59
    "log start time" <- w60
    n51 = Divide(x=u32 1000 ("milliseconds to wait"), y="Sample Rate (Hz)") -> (x/y=w62:dbl)
    n52 = Unbundle By Name(w44) -> ("TC0"=→"T7":dbl, "TC1"=→"T8":dbl, "TC2"=→"T9":dbl, "TC3"=→"T10":dbl, "TC4"=→"T11":dbl, "TC5"=→"T12":dbl)
    n53 = property on="error" class="Clust (strict)"("Visible"=w121) -> ()  [unwired: 2 in, 2 out]
    n54 = To Long Integer(number=w62) -> (32bit integer=w61:i32)
    n55 = Wait (ms)(milliseconds to wait=w61) -> ()  [unwired: 1 out]
    n56 = Select(t=state-enum."reset", s="Reset", f=w89) -> (s? t:f=w88:T3)
    n57 = call "loop-timer.vi"("loop-time-in"=w68) -> ("Loop Time (mS)"=→"Loop Time (mS)":u32, "loop-time-out"=w67:u32, "Hz"=→"Hz":dbl)  [unwired: 8 in]
    n58 = Unbundle By Name(w71) -> ("status"=→"Error Detected":bool)
    n59 = property on="Log Filepath Selection" class="Clust (strict)"("DisabledEnum"=w76) -> ()  [unwired: 2 in, 2 out]
    n60 = Select(t=state-enum."stop", s="Stop ADAM", f=w88) -> (s? t:f=w98:T3)
    n61 = Unbundle By Name(w45) -> ("TC0"=→"T1":dbl, "TC1"=→"T2":dbl, "TC2"=→"T3":dbl, "TC3"=→"T4":dbl, "TC4"=→"T5 (Ambi)":dbl, "TC5"=→"T6 (Airgap)":dbl)
    n62 = Cluster To Array(cluster=w44) -> (array=w47:dbl[])
    n63 = Select(t=state-enum."exit", s="exit", f=w98) -> (s? t:f=w101:T3)
    n64 = property on="Status Indicators" class="Clust (strict)"("Visible"="Debug Mode") -> ()  [unwired: 2 in, 2 out]
    n65 = property on="cmd-response" class="Clust (strict)"("Visible"="Debug Mode") -> ()  [unwired: 2 in, 2 out]
    n66 = Array Subset(array=w47, length=4) -> ()  [unwired: 1 in, 1 out]
    n67 = Cluster To Array(cluster=w45) -> (array=w49:dbl[])
    n68 = Array Subset(array=w49, length=4) -> ()  [unwired: 1 in, 1 out]
    n69 = property on="TC1:4 Zero point offset" class="Clust (strict)"("Visible"="Calibration") -> ()  [unwired: 2 in, 2 out]
    n70 = property on="TC5:8 Zero Point Offset" class="Clust (strict)"("Visible"="Calibration") -> ()  [unwired: 2 in, 2 out]
    "Loop Counter" <- w122
    "Program State" <- w84
  }
  n71 = flat-sequence {
    tunnel: w20 -> [w307]
    tunnel: w19 -> [w306]
    tunnel: [w305] -> w18
    tunnel: [w304] -> w17
    tunnel: w2 -> [w303]
    tunnel: [w302] -> w1
    tunnel: [w320] -> w23
    tunnel: w18 -> [w319]
    tunnel: w17 -> [w318]
    tunnel: w1 -> [w316]
    tunnel: w23 -> [w326]
    frame #0 {
      (unwired) T13 {"DO0"=FALSE, "DO1"=FALSE, "DO2"=FALSE, "DO3"=FALSE, "DO4"=FALSE, "DO5"=FALSE, "DO6"=FALSE, "DO7"=FALSE} ("5:Digital Outputs")
      n72 = case shown="True" w303 {
        selector: w303 -> [w308 w311]
        tunnel: w307 -> [w310 w315]
        tunnel: w306 -> [w309 w314]
        tunnel: [w309 w313] -> w305
        tunnel: [w310 w312] -> w304
        tunnel: [w308 w311] -> w302
        frame False {
        }
        frame True {
          n73 = call "adam5000-close-all.vi"("VISA Refnum in"=w315, "error in (no error)"=w314) -> ("VISA Refnum out"=w312:refnum<visa-resource-name>, "error out"=w313:errorcluster)  [unwired: 10 in, 2 out]
        }
      }
    }
    frame #1 {
      n74 = case shown="True" w316 {
        tunnel: [w321 w324] -> w320
        tunnel: w319 -> [w321 w323]
        tunnel: w318 -> [_ w322]
        frame False {
        }
        frame True {
          n75 = call "adam5000-stop-visa.vi"("error in (no error)"=w323, "VISA resource in"=w322) -> ("error out"=w324:errorcluster)  [unwired: 9 in]
        }
      }
      n76 = property on="Chassis Settings" class="Clust (strict)"("DisabledEnum"=T18."Enabled" ("Disabled")) -> ()  [unwired: 2 in, 2 out]
    }
    frame #2 {
      n77 = Merge Errors(w326) -> (w325:errorcluster)
      n78 = local write "error"(w325) -> ()
      n79 = Wait (ms)(milliseconds to wait=u32 500) -> ()  [unwired: 1 out]
    }
    frame #3 {
      # "Quit Labview"
      n80 = disable-structure "Conditional Disable Structure" shown="RUN_TIME_ENGINE==True" {
        frame condition #0 (active) {
        }
        frame condition #1 {
          # "Call Quit LabVIEW if running as a built application."
          n81 = Quit LabVIEW() -> ()  [unwired: 1 in]
        }
      }
    }
  }
